vi "Python executable does not exist--error.vi"() -> (0 "error out":errorcluster)   [LabVIEW 2026]
doc: "Python Executable does not exist."
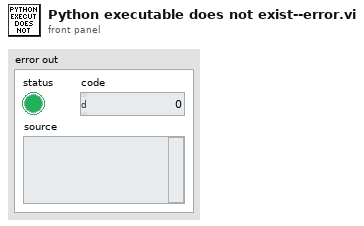
[diagram p1: front panel]
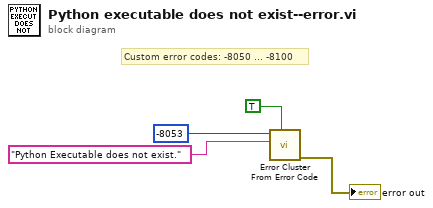
[diagram p0: block diagram]
diagram:
  # "Custom error codes: -8050 ... -8100"
  n1 = call <vilib>:"Error Cluster From Error Code.vi"("show call chain? (False)"=TRUE, "error message (\"\")"="Python Executable does not exist." ("error message (\"\")"), "error code (0)"=-8053) -> ("error out"=→"error out":errorcluster)  [unwired: 6 in]
